vi "VIH HelpGen - Palette - Get All Items.vi"(8 "error in":errorcluster, 9 "Entire hierarchy (T)":bool=TRUE, 10 "Include master menu (T)":bool=TRUE, 11 "Palette Path":path) -> (0 "error out":errorcluster, 2 "Items Array":T1[](array[typedef]), 3 "dup Palette Path":path)   [LabVIEW 2014]
doc: "::: VI Helpeks :::\nCopyright (c) 2000-2026 Konstantin Shifershteyn. All rights reserved."
uses:
  VIH HelpGen Typedef - Palette - Item Info Cluster.ctl
  VIH HelpGen Typedef - Palette - Item Type Enum.ctl
panel:
  # "VI Helpeks\nCopyright (c) 2012-2026 Konstantin Shifershteyn"
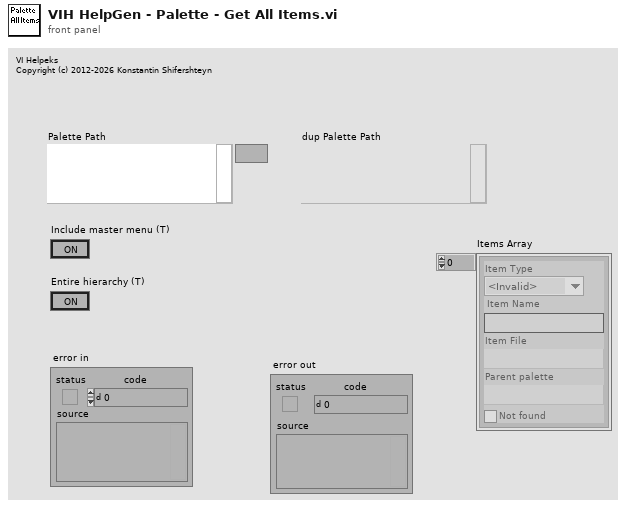
[diagram p1: front panel]
types:
  T1 = typedef "VIH HelpGen Typedef - Palette - Item Info Cluster.ctl" = cluster{"Item Type":T2, "Item Name":string, "Item File":path, "Parent palette":path, "Not found":bool}
  T2 = typedef "VIH HelpGen Typedef - Palette - Item Type Enum.ctl" = enum32{"<Invalid>", "<unknown>", "VI", "Menu", "LV Func", "Express VI", "Poly VI", "CTL", "HTML"}
  T3 = typedef "Palette Menu.lvlib/Palette Data.ctl" = cluster{"display name":string, "view format":T4, "palette width":i16, "items":T5, "256 color icon":picture, "B&W color icon":picture, "help information":T7, "palette description":string, "synchronize information":T8}
  T4 = typedef "Palette Menu.lvlib/View Format.ctl" = u16
  T5 = typedef "Palette Menu.lvlib/Items.ctl" = T6[]
  T6 = typedef "Palette Menu.lvlib/Item.ctl" = cluster{"item path":path, "library path (.lvlib)":path, "use default lvlib palette":bool, "short name":string, "place VI contents":bool, "hide synchronized item":bool, "reserve spot for synch item":bool, "configure when placing VI contents":bool}
  T7 = typedef "Palette Menu.lvlib/Help Info.ctl" = cluster{"help tag":string, "help file path ":path}
  T8 = typedef "Palette Menu.lvlib/Synchronize Info.ctl" = cluster{"synchronize with directory":bool, "synchronize directory path":path}
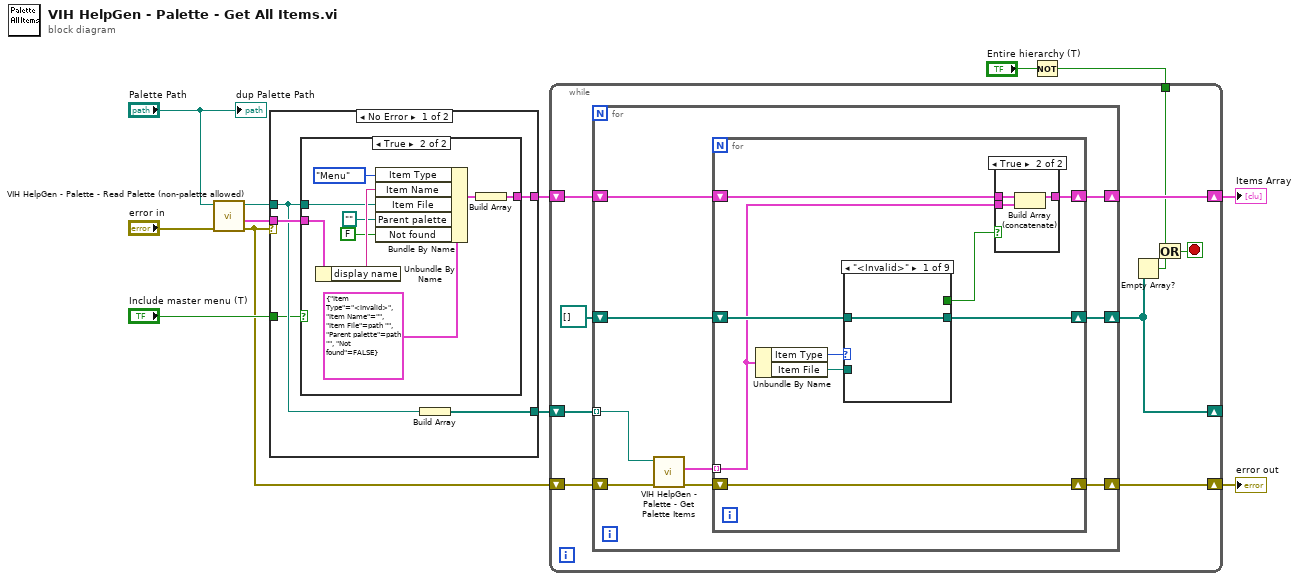
[diagram p0: block diagram]
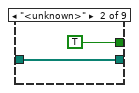
[diagram p4: hidden frame]
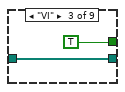
[diagram p5: hidden frame]
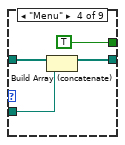
[diagram p6: hidden frame]
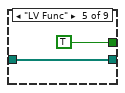
[diagram p7: hidden frame]
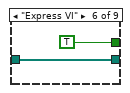
[diagram p8: hidden frame]
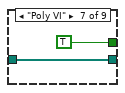
[diagram p9: hidden frame]
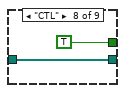
[diagram p10: hidden frame]
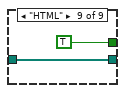
[diagram p11: hidden frame]
diagram:
  n1 = call "VIH HelpGen - Palette - Read Palette (non-palette allowed).vi"("error in"="error in", "Palette Path"="Palette Path") -> ("error out"=w3:errorcluster, "palette data"=w1:T3, "dup Palette Menu Path"=w2:path)  [unwired: 7 in]
  n2 = case shown="No Error" w3 {
    tunnel: [w17 _] -> w12
    tunnel: w1 -> [w16 _]
    tunnel: w2 -> [w15 _]
    tunnel: [w14 _] -> w9
    tunnel: "Include master menu (T)" -> [w13 _]
    frame No Error {
      n3 = case shown="True" w13 {
        tunnel: w16 -> [_ w24]
        tunnel: w15 -> [_ w21]
        tunnel: [_ w19] -> w14
        frame False {
        }
        frame True {
          n4 = Unbundle By Name(w24) -> ("display name"=w23:string)
          n5 = Bundle By Name(cluster=T1 {"Item Type"=enum."<Invalid>", "Item Name"="", "Item File"=path "", "Parent palette"=path "", "Not found"=FALSE} ("Item Info"), "Item Type"=VIH_HelpGen_Typedef_-_Palette_-_Item_Type_Enum."Menu", "Item Name"=w23, "Item File"=w21, "Parent palette"=path "", "Not found"=FALSE) -> (w20:T1)
          n6 = Build Array(w20) -> (w19:T1[])
        }
      }
      n7 = Build Array(w15) -> (w17:path[])
    }
    frame Error {
    }
  }
  n8 = Not(x="Entire hierarchy (T)") -> (.not. x?=w6:bool)
  n9 = while {
    shift-right: [w33] -> _
    shift-left: w12 -> [w36]
    shift-right: [w34] -> w11
    shift-left: w9 -> [w35]
    shift-right: [w31] -> w10
    shift-left: w3 -> [w32]
    tunnel: w6 -> [w29]
    stop <- w27 stop-if-true
    n10 = for {
      tunnel: w36 -> [w40] mode=indexing
      shift-right: [w41] -> w34
      shift-left: w35 -> [w42]
      shift-right: [w44] -> w33
      shift-left: path[] [] -> [w45]
      shift-right: [w43] -> w31
      shift-left: w32 -> [w39]
      n11 = call "VIH HelpGen - Palette - Get Palette Items.vi"("error in"=w39, "Palette Path"=w40) -> ("error out"=w37:errorcluster, "Items Array"=w38:T1[])  [unwired: 7 in, 1 out]
      n12 = for {
        shift-right: [w47] -> w44
        shift-left: w45 -> [w50]
        shift-right: [w54] -> w43
        shift-left: w37 -> [w54]
        shift-right: [w52] -> w41
        shift-left: w42 -> [w53]
        tunnel: w38 -> [w46] mode=indexing
        n13 = Unbundle By Name(w46) -> ("Item Type"=w51:T2, "Item File"=w49:path)
        n14 = case shown="\"<Invalid>\"" w51 {
          tunnel: w50 -> [w55 w57 w58 w63 w64 w66 w68 w70 w72]
          tunnel: w49 -> [_ _ _ w62 _ _ _ _ _]
          tunnel: [w55 w57 w58 w60 w64 w66 w68 w70 w72] -> w47
          tunnel: [_ TRUE TRUE TRUE TRUE TRUE TRUE TRUE TRUE] -> w48
          frame "<Invalid>" {
          }
          frame "<unknown>" {
          }
          frame "VI" {
          }
          frame "Menu" {
            n15 = Build Array (concatenate)(w63, w62) -> (w60:path[])
          }
          frame "LV Func" {
          }
          frame "Express VI" {
          }
          frame "Poly VI" {
          }
          frame "CTL" {
          }
          frame "HTML" {
          }
        }
        n16 = case shown="True" w48 {
          tunnel: w53 -> [w74 w77]
          tunnel: w46 -> [_ w76]
          tunnel: [w74 w75] -> w52
          frame False {
          }
          frame True {
            n17 = Build Array (concatenate)(w77, w76) -> (w75:T1[])
          }
        }
      }
    }
    n18 = Empty Array?(array=w33) -> (empty?=w28:bool)
    n19 = Or(x=w29, y=w28) -> (x .or. y?=w27:bool)
  }
  "Items Array" <- w11
  "error out" <- w10
  "dup Palette Path" <- "Palette Path"
